vi "Init.vi"(8 "error in (no error)":errorcluster, 11 "DAQNavi_AO in":refnum<class "DAQNavi_AO.lvclass">) -> (0 "error out":errorcluster, 3 "DAQNavi_AO out":refnum<class "DAQNavi_AO.lvclass">)   [LabVIEW 2021, in "DAQNavi_AO.lvclass"]
uses:
  DAQNavi_AO.lvclass
  DAQNavi_AO.lvclass/DAQNavi_AO.ctl
  <userlib>/DAQNavi Polymorphic VI/create/DAQNavi Create Channel(AO-Voltage).vi
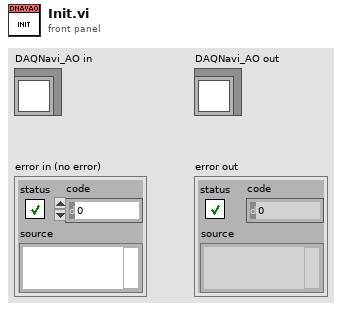
[diagram p1: front panel]
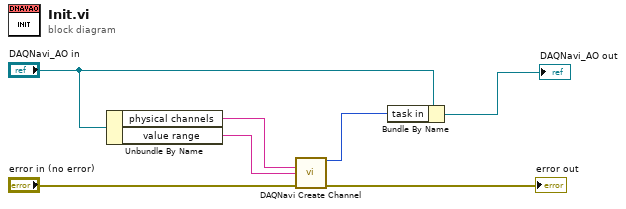
[diagram p0: block diagram]
diagram:
  n1 = Unbundle By Name("DAQNavi_AO in") -> ("physical channels"=w7:string, "value range"=w6:string)
  n2 = call-poly <userlib>:"DAQNavi Create Channel.vi"("physical channels"=w7, "value range"=w6, "error in (no error)"="error in (no error)") -> ("task out"=w5:i32, "error out"=→"error out":errorcluster)  [unwired: 11 in]
  n3 = Bundle By Name(cluster="DAQNavi_AO in", "task in"=w5) -> (→"DAQNavi_AO out":refnum<class "DAQNavi_AO.lvclass">)
